vi "remove_item_by_name.vi"(8 "error in (no error)":errorcluster, 10 "item_name":string, 11 "Table in":refnum<class "Table.lvclass">) -> (0 "error out":errorcluster, 2 "removed?":bool, 3 "Table out":refnum<class "Table.lvclass">)   [LabVIEW 2020, in "toml_edit.lvlib" / "Table.lvclass"]
uses:
  Table.lvclass
  Table.lvclass/Table.ctl
  dragon_toml_64.dll
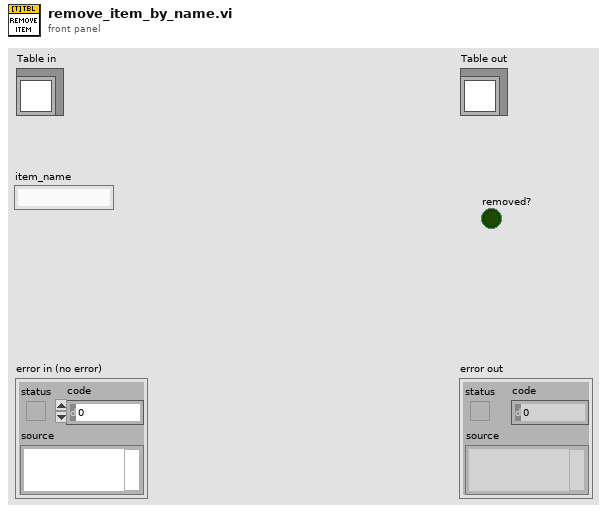
[diagram p1: front panel]
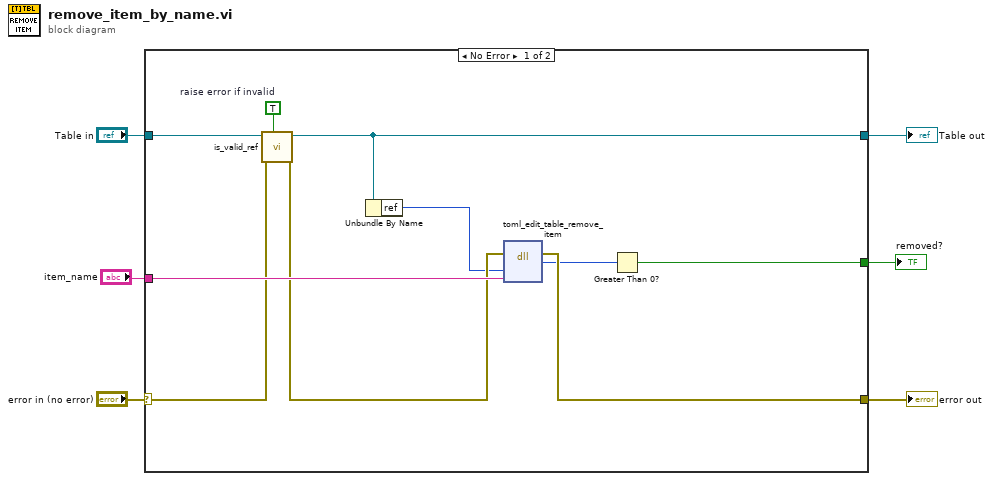
[diagram p0: block diagram]
diagram:
  n1 = case shown="No Error" "error in (no error)" {
    selector: "error in (no error)" -> [w11 w18]
    tunnel: [w15 w18] -> w5
    tunnel: [w13 w17] -> w3
    tunnel: "Table in" -> [w12 w17]
    tunnel: "item_name" -> [w16 _]
    tunnel: [w14 _] -> w1
    frame No Error {
      w9 = TRUE  # raise error if invalid
      n2 = call-dynamic "is_valid_ref.vi"("raise error if invalid? (False)"=w9, "error in (no error)"=w11, "Table in"=w12) -> ("error out"=w10:errorcluster, "Table out"=w13:refnum<class "Table.lvclass">)  [unwired: 6 in, 1 out]
      n3 = Unbundle By Name(w13) -> ("ref"=w8:u64)
      n4 = dll-call lib="C:/projects/dragon-desktop/source/submodules/toml-edit-labview/lv_src/dragon_toml_*.*" fn="toml_edit_table_remove_item"(error in=w10, "table_ref"=w8, "item_name"=w16) -> (error out=w15:errorcluster, "return"=w7:u64)  [unwired: 4 in, 1 out]
      n5 = Greater Than 0?(x=w7) -> (x > 0?=w14:bool)
    }
    frame Error {
    }
  }
  "error out" <- w5
  "Table out" <- w3
  "removed?" <- w1
